vi "Vibration Magnitude.vi"(10 "a_n-1":dbl, 11 "a_n":dbl) -> (2 "Settled (vm<0.1)":bool, 3 "vm":dbl)   [LabVIEW 2026]
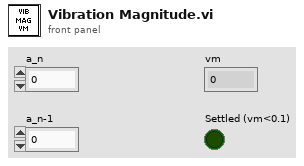
[diagram p1: front panel]
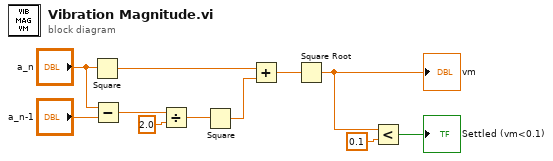
[diagram p0: block diagram]
diagram:
  n1 = Square(x="a_n") -> (x^2=w5:dbl)
  n2 = Subtract(x="a_n", y="a_n-1") -> (x-y=w9:dbl)
  n3 = Divide(x=w9, y=2.0) -> (x/y=w7:dbl)
  n4 = Square(x=w7) -> (x^2=w6:dbl)
  n5 = Add(x=w5, y=w6) -> (x+y=w4:dbl)
  n6 = Square Root(x=w4) -> (sqrt(x)=w3:dbl)
  "vm" <- w3
  n7 = Less?(x=w3, y=0.1) -> (x < y?=→"Settled (vm<0.1)":bool)
